vi "Create Workspace Ring Channel.vi"(8 "error in (no error)":errorcluster, 10 "Enum":variant, 11 "Channel Ref in":T1 format="%.0x") -> (0 "error out":errorcluster, 3 "Channel Ref out":T1 format="%.0x")   [LabVIEW 2020, in "FPGA Addon System Explorer.lvlib"]
uses:
  FPGA Addon System Explorer.lvlib
  <vilib>/NI VeriStand/Custom Device API/Custom Device Item Ref.ctl
  <vilib>/NI VeriStand/Custom Device API/Custom Device API.lvlib
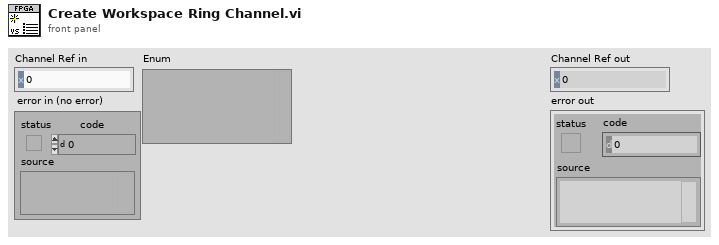
[diagram p1: front panel]
types:
  T1 = typedef "Custom Device API.lvlib/Custom Device Item Ref.ctl" = u64
  T2 = enum32{"invalid app kind", "Development System", "Run Time System", "Student Edition", "Embedded LabVIEW", "Evaluation", "Custom"}
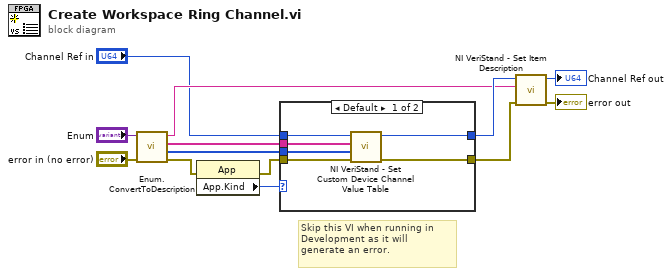
[diagram p0: block diagram]
diagram:
  # "Skip this VI when running in Development as it will generate an error."
  n1 = call "Enum.ConvertToDescription.vi"("error in (no error)"="error in (no error)", "Enum"="Enum") -> ("error out"=w3:errorcluster, "Number"=w12:i32[], "Values"=w13:string[], "Description"=w10:string)  [unwired: 6 in]
  n2 = property class="App"(error in=w3) -> (error out=w2:errorcluster, "App.Kind"=w1:T2)  [unwired: 1 in, 1 out]
  n3 = case shown="Default" w1 {
    tunnel: w13 -> [w19 _]
    tunnel: w12 -> [w18 _]
    tunnel: [w17 w21] -> w11
    tunnel: [w16 w20] -> w9
    tunnel: "Channel Ref in" -> [w15 w21]
    tunnel: w2 -> [w14 w20]
    frame Default {
      n4 = call <vilib>:"NI VeriStand - Set Custom Device Channel Value Table.vi"("error in (no error)"=w14, "Values"=w18, "Names"=w19, "Channel Ref in"=w15) -> ("error out"=w16:errorcluster, "Channel Ref out"=w17:T1)  [unwired: 6 in]
    }
    frame "Development System" {
    }
  }
  n5 = call <vilib>:"NI VeriStand - Set Item Description.vi"("error in (no error)"=w9, "Description"=w10, "Item Ref in"=w11) -> ("error out"=→"error out":errorcluster, "Item Ref out"=→"Channel Ref out":T1)  [unwired: 6 in, 1 out]
